vi "[ce] Get Lic Info.vi"(8 "error in":errorcluster, 11 "Lic (opt)":string) -> (0 "error out":errorcluster, 2 "CE License Info":T1)   [LabVIEW 2021]
doc: "::: CalcExpress Toolkit :::\nCopyright (c) 2000-2026 Konstantin Shifershteyn. All rights reserved."
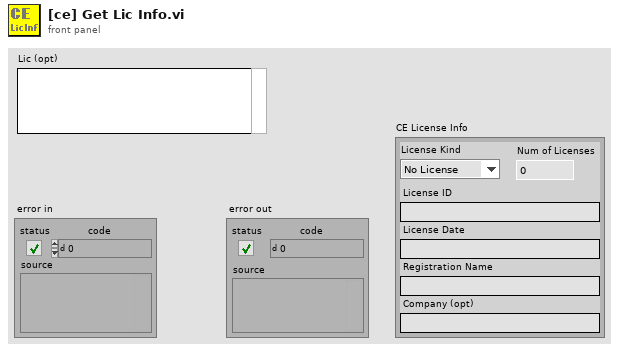
[diagram p1: front panel]
types:
  T1 = cluster{"License Kind":enum32{"No License", "Development", "Run-Time"}, "Num of Licenses":i32, "License ID":string, "License Date":string, "Registration Name":string, "Company (opt)":string}
  T2 = enum32{"invalid app kind", "Development System", "Run Time System", "Student Edition", "Embedded LabVIEW", "Evaluation", "Custom"}
  T3 = cluster{"License Kind":enum32{"No License", "Development", "Run-Time"}, "num":i32, string, string, string, string}
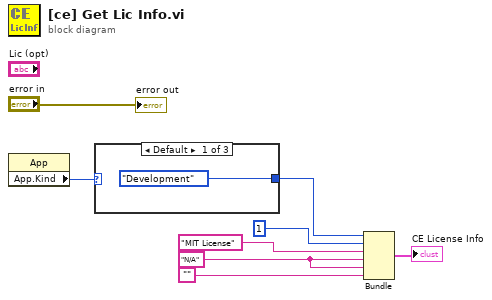
[diagram p0: block diagram]
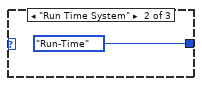
[diagram p2: hidden frame]
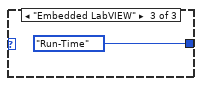
[diagram p3: hidden frame]
diagram:
  w5 = "N/A"
  n1 = property class="App"() -> ("App.Kind"=w4:T2)  [unwired: 2 in, 2 out]
  n2 = case shown="Default" w4 {
    tunnel: [enum32{"No License", "Development", "Run-Time"}."Development" ("License Kind") enum32{"No License", "Development", "Run-Time"}."Run-Time" ("License Kind") enum32{"No License", "Development", "Run-Time"}."Run-Time" ("License Kind")] -> w7
    frame Default {
    }
    frame "Run Time System" {
    }
    frame "Embedded LabVIEW" {
    }
  }
  n3 = Bundle("License Kind"=w7, "num"=1, "MIT License", w5, w5, "") -> (→"CE License Info":T3)  [unwired: 1 in]
  "error out" <- "error in"
